vi "Destroy.vi"(8 "error in (no error)":errorcluster, 11 "file handler in":refnum<class "File Handler.lvclass">) -> (0 "error out":errorcluster)   [LabVIEW 2018, in "GLog.lvlib" / "File Handler.lvclass"]
uses:
  File Handler.lvclass
  File Handler.lvclass/File Handler.ctl
panel:
  # "Connector Pane"
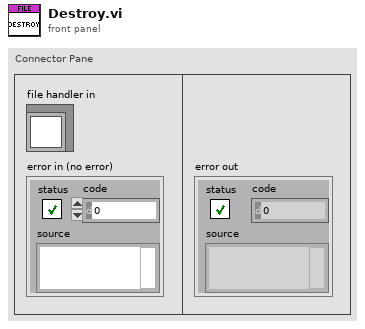
[diagram p1: front panel]
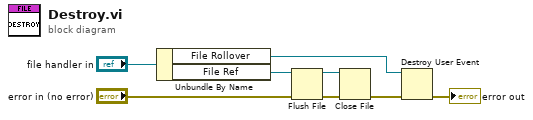
[diagram p0: block diagram]
diagram:
  n1 = Unbundle By Name("file handler in") -> ("File Rollover"=w1:refnum<user-event>, "File Ref"=w4:refnum<file>)
  n2 = Flush File(refnum=w4, error in="error in (no error)") -> (refnum out=w3:refnum<file>, error out=w5:errorcluster)
  n3 = Close File(refnum=w3, error in=w5) -> (error out=w6:errorcluster)  [unwired: 1 out]
  n4 = Destroy User Event(user event=w1, error in=w6) -> (error out=→"error out":errorcluster)
